vi "Show X Label.vi"(8 "error in (no error)":errorcluster, 9 "String":string, 10 "pixel center":cluster{"horizontal":i16, "vertical":i16}, 11 "Plot Bounds":T2) -> (0 "error out":errorcluster, 3 "new picture out":picture)   [LabVIEW 2025, in "XY Plotter.lvlib" / "XY Plotter.lvclass"]
uses:
  XY Plotter.lvclass
  <vilib>/Utility/miscctls.llb/LVRectTypeDef.ctl
panel:
  in  "font":T1={"Font Name"="Arial", "Size"=16, "Strikeout?"=FALSE, "Italic?"=FALSE, "Underline?"=FALSE, "Outline?"=FALSE, "Shadow?"=FALSE, "Bold?"=FALSE}
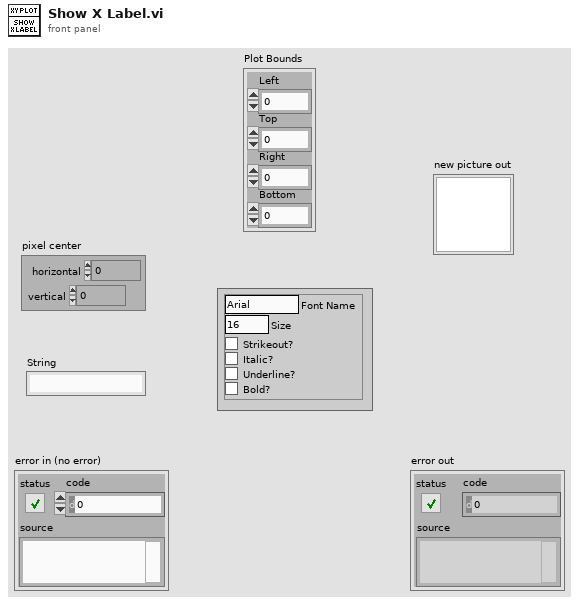
[diagram p1: front panel]
types:
  T1 = cluster{"Font Name":string, "Size":i16, "Strikeout?":bool, "Italic?":bool, "Underline?":bool, "Outline?":bool, "Shadow?":bool, "Bold?":bool}
  T2 = typedef "LVRectTypeDef.ctl" = cluster{"Left":i16, "Top":i16, "Right":i16, "Bottom":i16}
  T3 = enum16{"User-specified Font", "Application Font", "System Font", "Dialog Font"}
  T4 = cluster{"horizontal":enum16{"left", "center", "right"}, "vertical":enum16{"top", "center", "bottom"}}
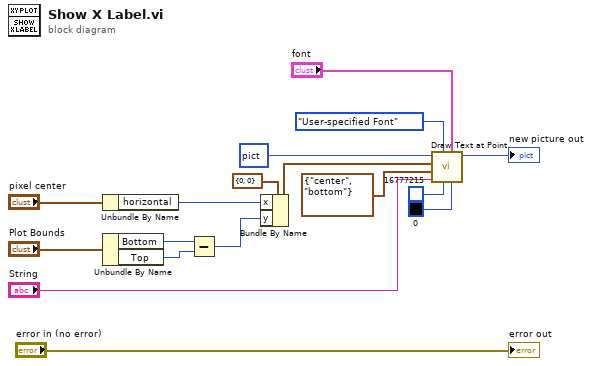
[diagram p0: block diagram]
diagram:
  n1 = Unbundle By Name("pixel center") -> ("horizontal"=w10:i16)
  n2 = Unbundle By Name("Plot Bounds") -> ("Bottom"=w4:i16, "Top"=w3:i16)
  n3 = Subtract(x=w4, y=w3) -> (x-y=w8:i16)
  n4 = Bundle By Name(cluster=cluster{"x":i16, "y":i16} {"x"=0, "y"=0} ("origin"), "x"=w10, "y"=w8) -> (w11:cluster{"x":i16, "y":i16})
  n5 = call <vilib>:"Draw Text at Point.vi"("BG color(transparent)"=u32 0, "[user-specified font]"="font", "text color(black)"=u32 16777215, "desired font(Application)"=T3."User-specified Font", "text"="String", "alignment(left, top)"=T4 {"horizontal"=enum."center", "vertical"=enum."bottom"}, "origin"=w11, "picture"=picture data[5B]) -> ("new picture"=→"new picture out":picture)  [unwired: 2 in, 1 out]
  "error out" <- "error in (no error)"
